vi "gainConvert (SubVI).vi"(8 "DACin":sgl, 9 "GainIN":sgl, 10 "GainSlope":sgl, 11 "GainOffset":sgl) -> (0 "GainOUT":sgl, 3 "DACout":dbl)   [LabVIEW 2017]
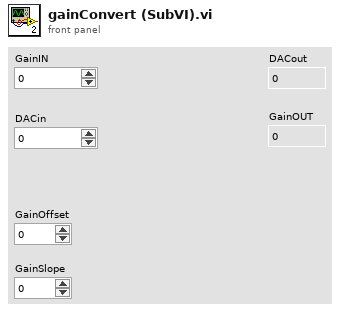
[diagram p1: front panel]
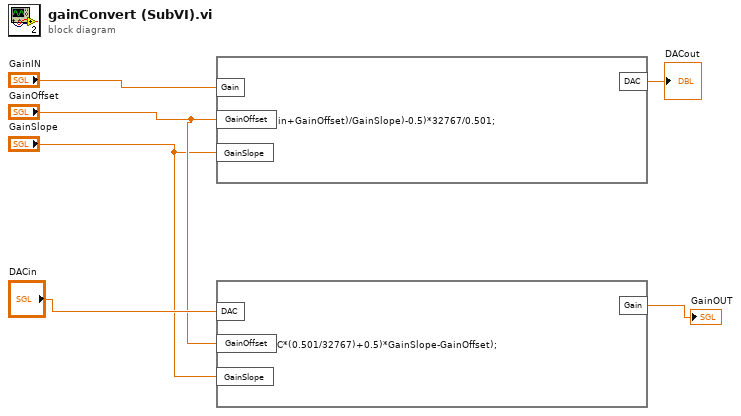
[diagram p0: block diagram]
diagram:
  n1 = formula code="DAC=(((Gain+GainOffset)/GainSlope)-0.5)*32767/0.501;"("Gain"="GainIN", "GainOffset"="GainOffset", "GainSlope"="GainSlope") -> ("DAC"=→"DACout":dbl)
  n2 = formula code="Gain=((DAC*(0.501/32767)+0.5)*GainSlope-GainOffset);"("DAC"="DACin", "GainOffset"="GainOffset", "GainSlope"="GainSlope") -> ("Gain"=→"GainOUT":dbl)
